vi "Create List.vi"(8 "error in (no error)":errorcluster, 9 "List type":i32(ring) items=["Number", "Bullet"], 10 "list elements":string[](array[string]), 11 "ooCalc in":refnum<class "ooCalc.lvclass">) -> (0 "error out":errorcluster, 2 "List":refnum<k24>, 3 "ooCalc out":refnum<class "ooCalc.lvclass">)   [LabVIEW 2009, in "ooCalc.lvclass"]
uses:
  ooCalc.lvclass
  C:/Projets/LAVAG/OpenOfficeRGT/AODL/DLLs/AODL.dll
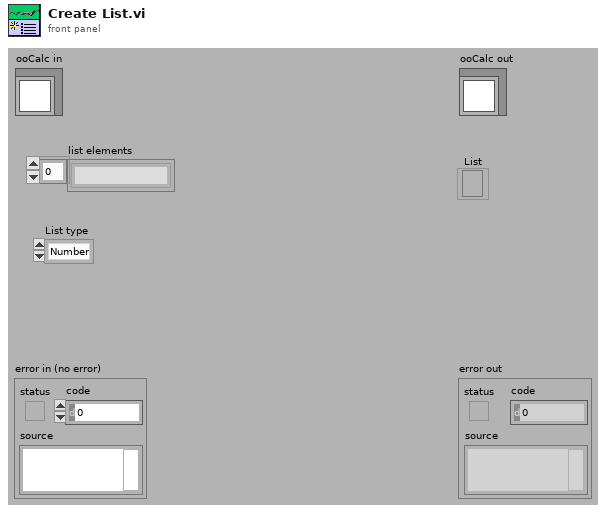
[diagram p1: front panel]
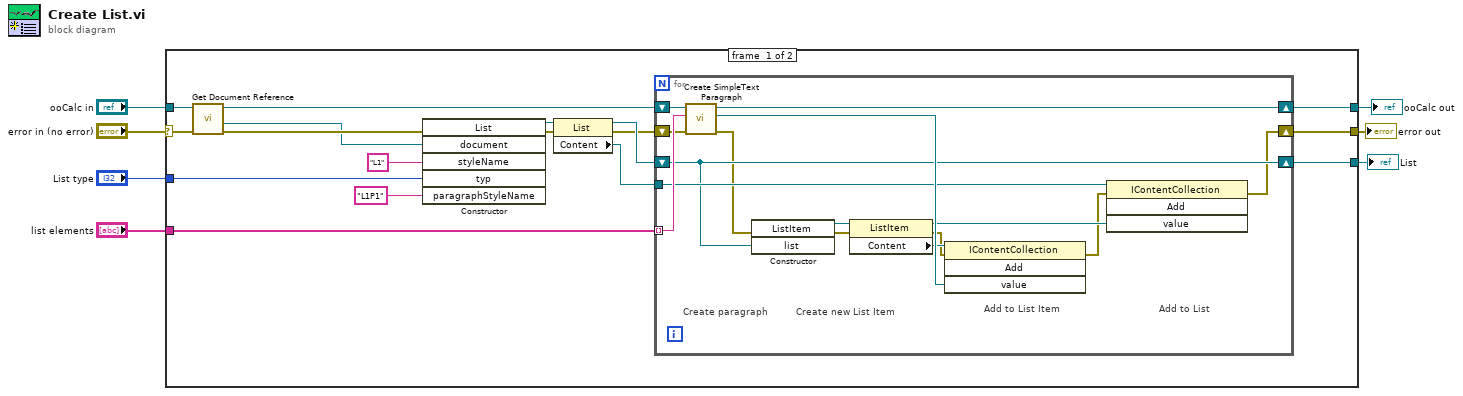
[diagram p0: block diagram]
diagram:
  n1 = case shown="No Error" "error in (no error)" {
    selector: "error in (no error)" -> [w10 w41]
    tunnel: [w15 w41] -> w6
    tunnel: [w14 w40] -> w4
    tunnel: "ooCalc in" -> [w12 w40]
    tunnel: "List type" -> [w17 _]
    tunnel: "list elements" -> [w16 _]
    tunnel: [w13 _] -> w1
    frame #0 {
      n2 = call-dynamic "Get Document Reference.vi"("error in (no error)"=w10, "ooDocument in"=w12) -> ("error out"=w9:errorcluster, "Document"=w8:refnum<k24>, "ooDocument out"=w11:refnum<class "ooCalc.lvclass">)  [unwired: 7 in]
      n3 = constructor class="List"(error in=w9, "document"=w8, "styleName"="L1", "typ"=w17, "paragraphStyleName"="L1P1") -> (reference out=w20:refnum<k24>, error out=w19:errorcluster)  [unwired: 2 in, 5 out]
      n4 = property class="List"(reference=w20, error in=w19) -> (reference out=w21:refnum<k24>, error out=w18:errorcluster, "Content"=w22:refnum<k24>)
      n5 = for {
        tunnel: w16 -> [w38] mode=indexing
        shift-right: [w37] -> w14
        shift-left: w11 -> [w39]
        tunnel: w22 -> [w33]
        shift-right: [w30] -> w13
        shift-left: w21 -> [w30]
        shift-right: [w28] -> w15
        shift-left: w18 -> [w25]
        # "Add to List"
        # "Create new List Item"
        # "Add to List Item"
        # "Create paragraph"
        n6 = call-dynamic "Create SimpleText Paragraph.vi"("error in (no error)"=w25, "simpleText"=w38, "ooCalc in"=w39) -> ("error out"=w26:errorcluster, "SimpleTextParagraph"=w36:refnum<k24>, "ooCalc out"=w37:refnum<class "ooCalc.lvclass">)  [unwired: 6 in]
        n7 = constructor class="ListItem"(error in=w26, "list"=w30) -> (reference out=w35:refnum<k24>, error out=w29:errorcluster)  [unwired: 2 in, 2 out]
        n8 = property class="ListItem"(reference=w35, error in=w29) -> (reference out=w32:refnum<k24>, error out=w27:errorcluster, "Content"=w34:refnum<k24>)
        n9 = invoke class="IContentCollection" method="Add"(reference=w34, error in=w27, "value"=w36) -> (error out=w31:errorcluster)  [unwired: 1 in, 3 out]
        n10 = invoke class="IContentCollection" method="Add"(reference=w33, error in=w31, "value"=w32) -> (error out=w28:errorcluster)  [unwired: 1 in, 3 out]
      }
    }
    frame #1 {
    }
  }
  "error out" <- w6
  "ooCalc out" <- w4
  "List" <- w1
